vi "Actor.vi"(4 "Async Elements":refnum<class "Async Elements.lvclass">, 11 "TEMPLATE Actor in":refnum<class "TEMPLATE Actor.lvclass">) -> (0 "Error out":errorcluster, 3 "TEMPLATE Actor out":refnum<class "TEMPLATE Actor.lvclass">)   [LabVIEW 2020, in "_Template.lvlib" / "Templates.lvlib" / "TEMPLATE jettl Actor.lvlib" / "TEMPLATE Actor.lvlib" / "TEMPLATE Actor.lvclass"]
uses:
  TEMPLATE Actor.lvclass
  C:/git/jettl/src/jettl/jettl/Actor/Actor.lvclass
  jettl/jettl/Async Elements/Async Elements.lvclass
  TEMPLATE Refs/Refs.ctl
  TEMPLATE Refs/TEMPLATE Refs/TEMPLATE Refs.lvclass/TEMPLATE Refs.ctl
  jettl/jettl/Base Async Elements/Base Async Elements/Base Async Elements.lvclass/Base Async Elements.ctl
  jettl/jettl/Base Attributes/Base Attributes/Base Attributes.lvclass/Base Attributes.ctl
  jettl/jettl/Event Transport/Event Transport/Event Transport.lvclass/Event Transport.ctl
  jettl/jettl/Event Transport/Read Msg Ref.vi
  jettl/jettl/Event Transport/Event Transport/Init Transport.vi
  jettl/jettl/Update Attributes A.vi
  jettl/jettl/Update Attributes B.vi
  jettl/jettl/Base Async Elements/Read Async Elements.vi
  jettl/jettl/Event Transport/Event Transport/Read Msg Ref.vi
  jettl/jettl/Base Attributes/Init Attributes.vi
  jettl/jettl/Base Async Elements/Base Async Elements/Read Async Elements.vi
  jettl/jettl/Base Attributes/Base Attributes/Init Attributes.vi
  TEMPLATE Refs/TEMPLATE Refs/TEMPLATE Refs.lvclass
  C:/git/jettl/src/jettl/jettl/Refs/Refs.lvclass
  jettl/jettl/Event Transport/Event Transport/Event Transport.lvclass
  C:/git/jettl/src/jettl/jettl/Transport/Transport.lvclass
  jettl/jettl/Base Attributes/Base Attributes/Base Attributes.lvclass
  C:/git/jettl/src/jettl/jettl/Attributes/Attributes.lvclass
  jettl/jettl/Call.vi
  jettl/jettl/Stop jettl Msg/Stop/Stop.vi
  jettl/jettl/Stop jettl Msg/Stop/Call.vi
  jettl/jettl/Attributes/Attributes.lvclass
  jettl/jettl/Base Async Elements/Base Async Elements/Base Async Elements.lvclass
  jettl/jettl/Msg/Msg.lvclass
  jettl/jettl/Actor/Actor.lvclass
  jettl/jettl/Transport/Transport.lvclass
  TEMPLATE Refs/TEMPLATE Refs.lvlib
  jettl/jettl/jettl.lvlib
  jettl/jettl/Event Transport/Event Transport.lvlib
panel:
  # "This panel can be extended with controls and indicators, though do not modify the conn pane."
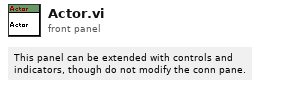
[diagram p1: front panel]
types:
  T1 = typedef "_Template.lvlib/Templates.lvlib/TEMPLATE jettl Actor.lvlib/TEMPLATE Actor.lvlib/TEMPLATE Refs.lvlib/Refs.ctl" = cluster{"placeholder":refnum<vi>}
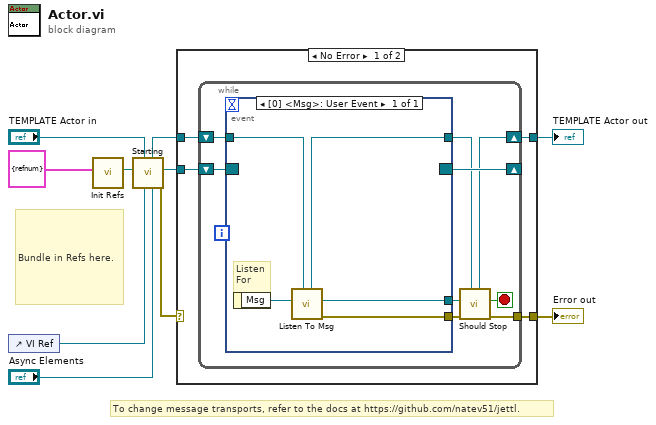
[diagram p0: block diagram]
diagram:
  # "To change message transports, refer to the docs at https://github.com/natev51/jettl."
  # "Bundle in Refs here."
  n1 = control-ref of="VI Ref"() -> (w3:refnum<vi>)
  n2 = call "Init Refs.vi"("Refs"=T1 {"placeholder"=refnum} ("Control Refs")) -> ("Refs"=w4:refnum<class "Refs.lvclass">)  [unwired: 10 in]
  n3 = call "Starting.vi"("Async Elements"="Async Elements", "VI Ref"=w3, "Actor in"="TEMPLATE Actor in", "Refs"=w4) -> ("Error out"=w5:errorcluster, "Msg Ref"=w2:refnum<event-registration>, "Actor out"=w6:refnum<class "TEMPLATE Actor.lvclass">)  [unwired: 5 in]
  n4 = case shown="No Error" w5 {
    selector: w5 -> [_ w29]
    tunnel: [w11 w30] -> w9
    tunnel: w6 -> [w13 w30]
    tunnel: [w14 w29] -> w10
    tunnel: w2 -> [w12 _]
    frame No Error {
      n5 = while {
        shift-right: [w16] -> w11
        shift-left: w13 -> [w22]
        tunnel: [w20] -> w14
        shift-right: [w17] -> _
        shift-left: w12 -> [w23]
        stop <- w19 stop-if-true
        n6 = event shown="[0] <Msg>: User Event" {
          selector: w23 -> [_]
          dyn-events: [_] -> w17
          timeout: _ -> [_]
          tunnel: w22 -> [w28]
          tunnel: [w26] -> w15
          tunnel: [w25] -> w21
          tunnel: [w24] -> w18
          event User Event {
            # "Listen\nFor"
            n7 = event-data() -> ("Msg"=w27:refnum<class "Msg.lvclass">)  [unwired: 1 in]
            n8 = call "Listen To Msg.vi"("Actor in"=w28, "Msg"=w27) -> ("Error out"=w25:errorcluster, "Msg Output"=w24:refnum<class "Msg Output.lvclass">, "Actor out"=w26:refnum<class "TEMPLATE Actor.lvclass">)  [unwired: 7 in]
          }
        }
        n9 = call "Should Stop.vi"("Actor in"=w15, "Error in"=w21, "Msg Output"=w18) -> ("Error out"=w20:errorcluster, "Stop"=w19:bool, "Actor out"=w16:refnum<class "TEMPLATE Actor.lvclass">)  [unwired: 6 in]
      }
    }
    frame Error {
    }
  }
  "TEMPLATE Actor out" <- w9
  "Error out" <- w10
